vi "Util_Trajectory_ReadFile.vi"(8 "error in (no error)":errorcluster, 11 "FileName":string="trajectory.csv") -> (0 "error out":errorcluster, 3 "outTRAJECTORY":T1 {"States"."POSE"."ROTATION"."SIN" format="%13.4f"; "States"."POSE"."ROTATION"."COS" format="%13.4f"; "States"."POSE"."ROTATION"."VALUE" format="%13.4f"; "States"."POSE"."TRANSLATION"."Y" format="%14.3f"; "States"."POSE"."TRANSLATION"."X" format="%14.3f"; "TotalTImeSecs" format="%20.3f"}, 4 "Full FIlename":string)   [LabVIEW 2019, in "Trajectory_Library.lvlib"]
doc: "Create a trajectory from a CSV file. This can be used on a PC or the RoboRIO. Normally the CSV file is created as output from one of the trajectory utility programs. The file could also be created manually or by a custom written program.\n\nParameters:\n - FileName -- Name of the CSV file to read. See file name notes for additional information.\n - Error In -- Input error cluster (optional)\n\nReturns:\n - outTrajectory - Trajectory data structure cluster\n - Error out - returned error cluster\n\nNotes on use:\n -- This routine writes informational messges to the console and to the driver station log.\n\nNotes on file naming:\n -- The file name must include the extention. \".csv\" is not automatically appended to the name. \n -- The file name can be a simple file or an absolute path. If a simple file name is used the default path on the RoboRIO is: \"home:\\lvuser\\natinst\\LabVIEW Data\". On a Windows PC the default path is the LabVIEW default directory. Normally this is: “%HOMEDRIVE%%HOMEPATH%\\Documents\\LabView Data\".\n -- Filenames on the RoboRIO, which runs Linux, are case sensitive.\n\nNotes on file contents:\n -- Blank lines are ignored.\n -- Lines that begin with either #, !, or ' in the first character are considered comments and are ignored. \n -- Other lines are interpretted as comma separated data as follows:\n -- Trajectory time -- seconds\n -- Expected velocity -- meters/sec\n -- Expected acceleration -- meters/sec^2\n -- Expected X position -- meters\n -- Expected Y position -- meters\n -- Expected heading (not necessarily robot orientation) -- radians\n -- Expected curvature (rotational portion of velocity) -- radians/meter\n -- Optional comment string. This ignored when reading file"
uses:
  Trajectory_Library.lvlib
  TypeDef/TRAJECTORY.ctl
  TypeDef/TRAJ_STATE.ctl
  TypeDef/POSE2D.ctl
  TypeDef/TRANSLATION2D.ctl
  TypeDef/ROTATION2D.ctl
  <vilib>/Utility/error.llb/whitespace.ctl
  Rotation2d_CreateAngle.vi
  Translation2d_Create.vi
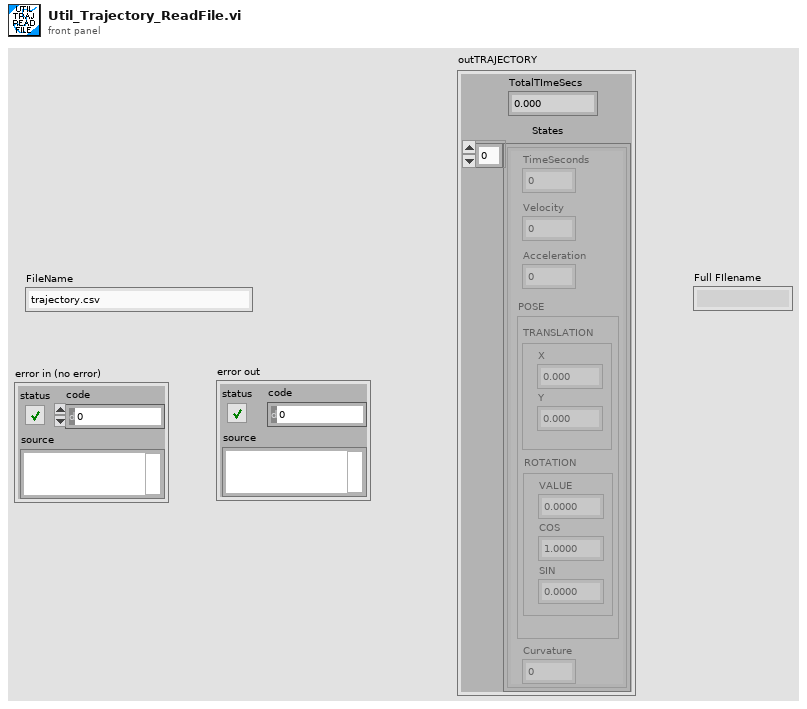
[diagram p1: front panel]
types:
  T1 = typedef "Trajectory_Library.lvlib/TRAJECTORY.ctl" = cluster{"TotalTImeSecs":dbl, "States":T2[]}
  T2 = typedef "Trajectory_Library.lvlib/TRAJ_STATE.ctl" = cluster{"TimeSeconds":dbl, "Velocity":dbl, "Acceleration":dbl, "POSE":T3, "Curvature":dbl}
  T3 = typedef "Trajectory_Library.lvlib/POSE2D.ctl" = cluster{"TRANSLATION":T4, "ROTATION":T5}
  T4 = typedef "Trajectory_Library.lvlib/TRANSLATION2D.ctl" = cluster{"X":dbl, "Y":dbl}
  T5 = typedef "Trajectory_Library.lvlib/ROTATION2D.ctl" = cluster{"VALUE":dbl, "COS":dbl, "SIN":dbl}
  T6 = enum16{"open", "replace", "create", "open or create", "replace or create", "replace or create with confirmation"}
  T7 = typedef "whitespace.ctl" = u16
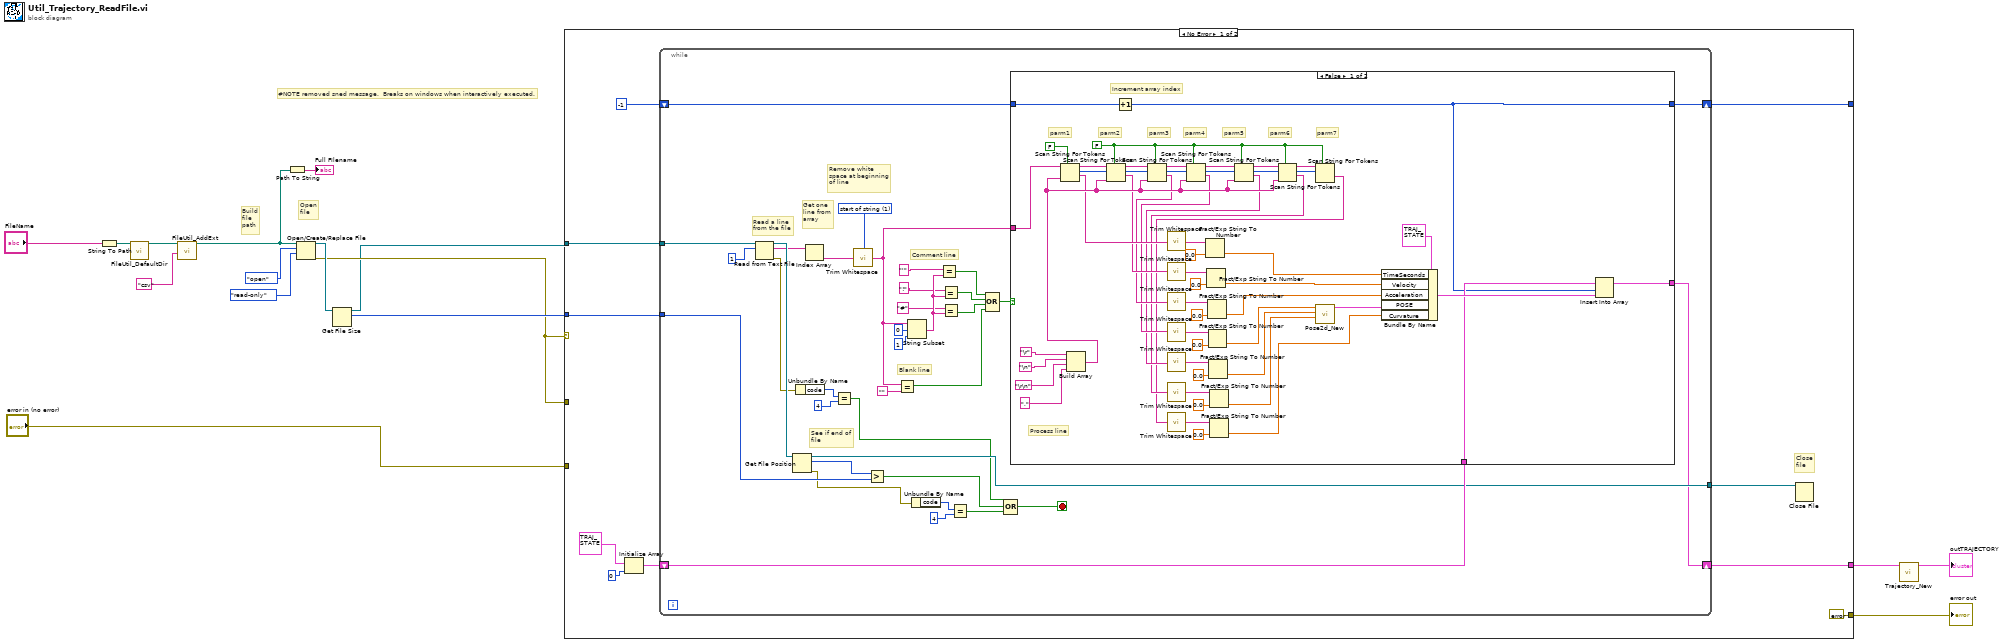
[diagram p0: block diagram]
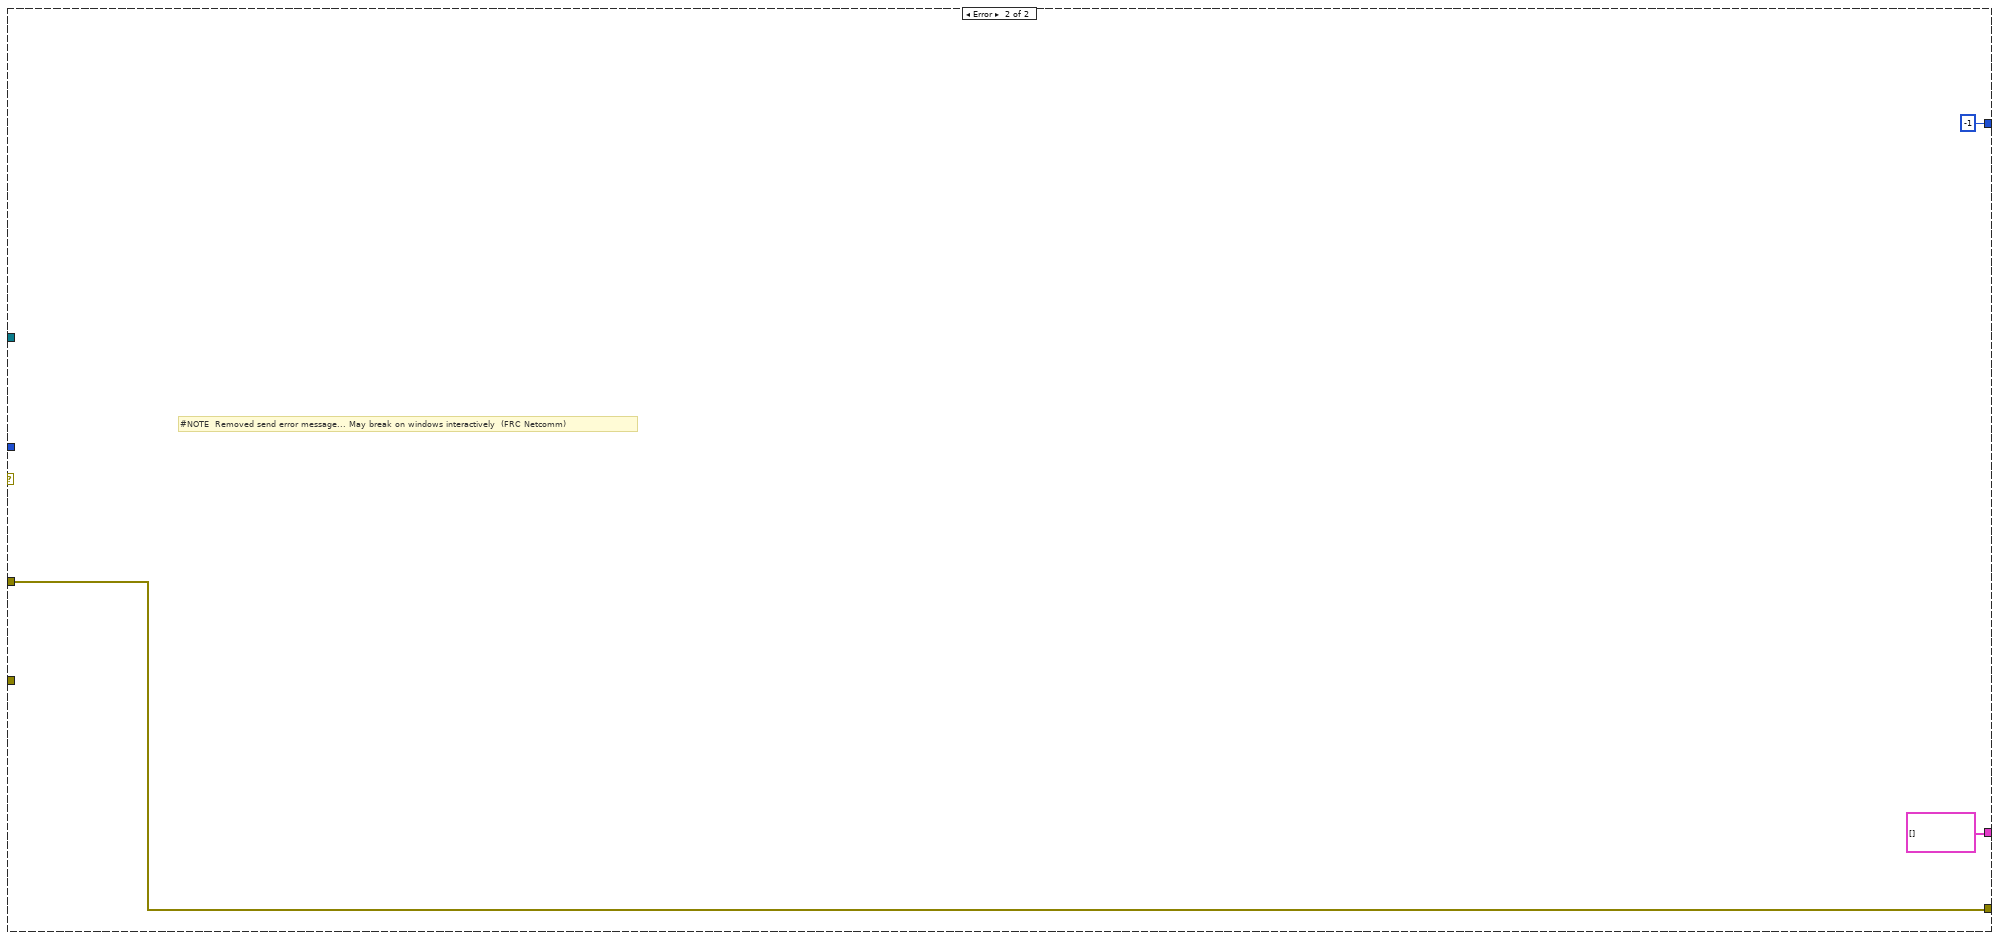
[diagram p3: hidden frame]
diagram:
  # "#NOTE removed sned message.  Breaks on windows when interactively executed."
  # "Open\nfile"
  # "Build\nfile\npath"
  n1 = String To Path(string="FileName") -> (path=w2:path)
  n2 = call "FileUtil_DefaultDir.vi"("Path in"=w2) -> ("Path Out"=w4:path)  [unwired: 10 in]
  n3 = call "FileUtil_AddExt.vi"("Extension"="csv", "Path in"=w4) -> ("Path out"=w1:path)  [unwired: 9 in]
  n4 = Path To String(path=w1) -> (string=→"Full FIlename":string)
  n5 = Open/Create/Replace File(file path (use dialog)=w1, operation (0:open)=T6."open", access (0:read/write)=enum16{"read/write", "read-only", "write-only"}."read-only") -> (refnum out=w14:refnum<file>, error out=w12:errorcluster)  [unwired: 3 in, 1 out]
  n6 = Get File Size(file=w14) -> (refnum out=w7:refnum<file>, size (in bytes)=w13:i64)  [unwired: 1 in, 1 out]
  n7 = case shown="No Error" w12 {
    tunnel: w7 -> [w26 _]
    tunnel: w13 -> [w24 _]
    tunnel: [w20 i16 -1] -> _
    tunnel: [w19 T2[] []] -> w11
    tunnel: w12 -> [_ w120]
    tunnel: [errorcluster {"status"=FALSE, "code"=0, "source"=""} ("error out") w120] -> w9
    tunnel: "error in (no error)" -> [_ _]
    frame No Error {
      # "Close\nfile"
      n8 = Initialize Array(T2 {"TimeSeconds"=0.0, "Velocity"=0.0, "Acceleration"=0.0, "POSE"={"TRANSLATION"={"X"=0.0, "Y"=0.0}, "ROTATION"={"VALUE"=0.0, "COS"=1.0, "SIN"=0.0}}, "Curvature"=0.0} ("TRAJ_STATE"), 0 ("dimension size")) -> (w21:T2[])
      n9 = while {
        tunnel: w26 -> [w62]
        tunnel: w24 -> [w58]
        tunnel: [w38] -> w23
        shift-right: [w28] -> w20
        shift-left: i16 -1 -> [w42]
        shift-right: [w27] -> w19
        shift-left: w21 -> [w40]
        stop <- w36 stop-if-true
        w57 = T7 1 items=["both", "start of string", "end of string"] ("location (both)")
        # "Comment line"
        # "Blank line"
        # "Remove white \nspace at beginning\nof line"
        # "Get one\nline from\narray"
        # "Read a line\nfrom the file"
        # "See if end of \nfile"
        n10 = Read from Text File(file (use dialog)=w62, count=1) -> (refnum out=w60:refnum<file>, text=w56:string[], error out=w39:errorcluster)  [unwired: 2 in, 1 out]
        n11 = Get File Position(7:w60) -> (0:w31:errorcluster, 2:w59:i64, 3:w38:refnum<file>)  [unwired: 1 in]
        n12 = Unbundle By Name(w39) -> ("code"=w35:i32)
        n13 = Index Array(array=w56) -> (element=w55:string)  [unwired: 1 in]
        n14 = Equal?(x=w35, y=4) -> (x = y?=w30:bool)
        n15 = call <vilib>:"Trim Whitespace.vi"("string"=w55, "location (both)"=w57) -> ("trimmed string"=w41:string)
        n16 = Greater?(x=w59, y=w58) -> (0:w37:bool)
        n17 = Equal?(x=w41, y="") -> (x = y?=w44:bool)
        n18 = String Subset(string=w41, offset (0)=0, length (rest)=1 ("length (rest)")) -> (substring=w51:string)
        n19 = Unbundle By Name(w31) -> ("code"=w33:i32)
        n20 = Equal?(x="'", y=w51) -> (x = y?=w47:bool)
        n21 = Equal?(x="!", y=w51) -> (x = y?=w46:bool)
        n22 = Equal?(x="#", y=w51) -> (x = y?=w45:bool)
        n23 = Equal?(x=w33, y=4) -> (x = y?=w29:bool)
        n24 = Compound Arithmetic op=OR(w47, w46, w45, w44) -> (w43:bool)
        n25 = Compound Arithmetic op=OR(w30, w37, w29) -> (w36:bool)
        n26 = case shown="False" w43 {
          tunnel: w42 -> [w117 w118]
          tunnel: [w80 w118] -> w28
          tunnel: w41 -> [w79 _]
          tunnel: w40 -> [w82 w119]
          tunnel: [w81 w119] -> w27
          frame False {
            w69 = FALSE ("allow empty tokens? (F)")
            # "parm6"
            # "parm7"
            # "parm5"
            # "parm4"
            # "parm3"
            # "parm2"
            # "parm1"
            # "Increment array index"
            # "Process line"
            n27 = Build Array("\r", "\n", "\r\n", ",") -> (w111:string[])
            n28 = Scan String For Tokens(5:FALSE ("allow empty tokens? (F)"), 6:w111, 9:w79) -> (1:w100:string, 2:w105:i32, 3:w110:string)  [unwired: 3 in, 1 out]
            n29 = Scan String For Tokens(5:w69, 6:w111, 8:w105, 9:w110) -> (1:w99:string, 2:w104:i32, 3:w109:string)  [unwired: 2 in, 1 out]
            n30 = Increment(x=w117) -> (x+1=w80:i16)
            n31 = Scan String For Tokens(5:w69, 6:w111, 8:w104, 9:w109) -> (1:w98:string, 2:w103:i32, 3:w108:string)  [unwired: 2 in, 1 out]
            n32 = call <vilib>:"Trim Whitespace.vi"("string"=w100) -> ("trimmed string"=w64:string)  [unwired: 1 in]
            n33 = call <vilib>:"Trim Whitespace.vi"("string"=w99) -> ("trimmed string"=w93:string)  [unwired: 1 in]
            n34 = call <vilib>:"Trim Whitespace.vi"("string"=w98) -> ("trimmed string"=w88:string)  [unwired: 1 in]
            n35 = Scan String For Tokens(5:w69, 6:w111, 8:w103, 9:w108) -> (1:w97:string, 2:w102:i32, 3:w107:string)  [unwired: 2 in, 1 out]
            n36 = call <vilib>:"Trim Whitespace.vi"("string"=w97) -> ("trimmed string"=w87:string)  [unwired: 1 in]
            n37 = Fract/Exp String To Number(string=w64, default (0 dbl)=0.0 ("default (0 DBL)")) -> (number=w65:dbl)  [unwired: 2 in, 1 out]
            n38 = Fract/Exp String To Number(string=w93, default (0 dbl)=0.0 ("default (0 DBL)")) -> (number=w84:dbl)  [unwired: 2 in, 1 out]
            n39 = Fract/Exp String To Number(string=w88, default (0 dbl)=0.0 ("default (0 DBL)")) -> (number=w77:dbl)  [unwired: 2 in, 1 out]
            n40 = Fract/Exp String To Number(string=w87, default (0 dbl)=0.0 ("default (0 DBL)")) -> (number=w75:dbl)  [unwired: 2 in, 1 out]
            n41 = Scan String For Tokens(5:w69, 6:w111, 8:w102, 9:w107) -> (1:w96:string, 2:w101:i32, 3:w106:string)  [unwired: 2 in, 1 out]
            n42 = call <vilib>:"Trim Whitespace.vi"("string"=w96) -> ("trimmed string"=w86:string)  [unwired: 1 in]
            n43 = Fract/Exp String To Number(string=w86, default (0 dbl)=0.0 ("default (0 DBL)")) -> (number=w74:dbl)  [unwired: 2 in, 1 out]
            n44 = Scan String For Tokens(5:w69, 6:w111, 8:w101, 9:w106) -> (1:w95:string, 2:w67:i32, 3:w68:string)  [unwired: 2 in, 1 out]
            n45 = call <vilib>:"Trim Whitespace.vi"("string"=w95) -> ("trimmed string"=w85:string)  [unwired: 1 in]
            n46 = Fract/Exp String To Number(string=w85, default (0 dbl)=0.0 ("default (0 DBL)")) -> (number=w73:dbl)  [unwired: 2 in, 1 out]
            n47 = Scan String For Tokens(5:w69, 8:w67, 9:w68) -> (1:w66:string)  [unwired: 3 in, 3 out]
            n48 = call <vilib>:"Trim Whitespace.vi"("string"=w66) -> ("trimmed string"=w71:string)  [unwired: 1 in]
            n49 = Fract/Exp String To Number(string=w71, default (0 dbl)=0.0 ("default (0 DBL)")) -> (number=w70:dbl)  [unwired: 2 in, 1 out]
            n50 = call "Pose2d_New.vi"("Heading"=w73, "Y"=w74, "X"=w75) -> ("out POSe"=w76:T3)  [unwired: 8 in]
            n51 = Bundle By Name(cluster=T2 {"TimeSeconds"=0.0, "Velocity"=0.0, "Acceleration"=0.0, "POSE"={"TRANSLATION"={"X"=0.0, "Y"=0.0}, "ROTATION"={"VALUE"=0.0, "COS"=1.0, "SIN"=0.0}}, "Curvature"=0.0} ("TRAJ_STATE"), "TimeSeconds"=w65, "Velocity"=w84, "Acceleration"=w77, "POSE"=w76, "Curvature"=w70) -> (w83:T2)
            n52 = Insert Into Array(array=w82, index=w80, new element=w83) -> (w81:T2[])
          }
          frame True {
            # "Comment -- ignore."
          }
        }
      }
      n53 = Close File(refnum=w23) -> ()  [unwired: 1 in, 2 out]
    }
    frame Error {
      # "#NOTE  Removed send error message... May break on windows interactively  (FRC Netcomm)"
    }
  }
  "error out" <- w9
  n54 = call "Trajectory_New.vi"("TRAJ_STATES"=w11) -> ("TRAJECTORY"=→"outTRAJECTORY":T1)  [unwired: 10 in]
